vi "test tool call default arguments.vi"(8 "error in (no error)":errorcluster) -> (0 "error out":errorcluster, 3 "body":string)   [LabVIEW 2020, in "MCP Server tests.lvlib"]
doc: "arguments is optional in tools/call. Without it the tool runs with the default values of its inputs: fake_tool_add answers with the sum 0, and the answer is a result, not an error."
uses:
  MCP Server tests.lvlib
  <vilib>/addons/_JKI Toolkits/Caraya/classes/Test/Test.lvclass
  <vilib>/JDP Science/JSONtext/JSONtext.lvlib
  a69b8a6d-5d8a-435b-aaad-afb045a32dc0.vi
  <vilib>/addons/_JKI Toolkits/Caraya/classes/Assert/Assert.lvclass
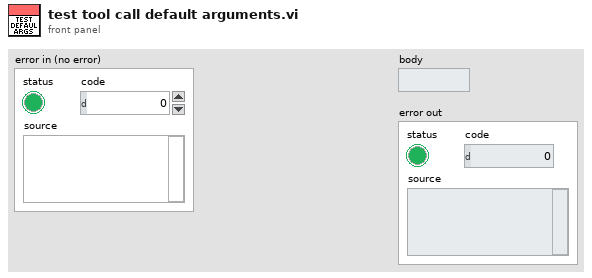
[diagram p1: front panel]
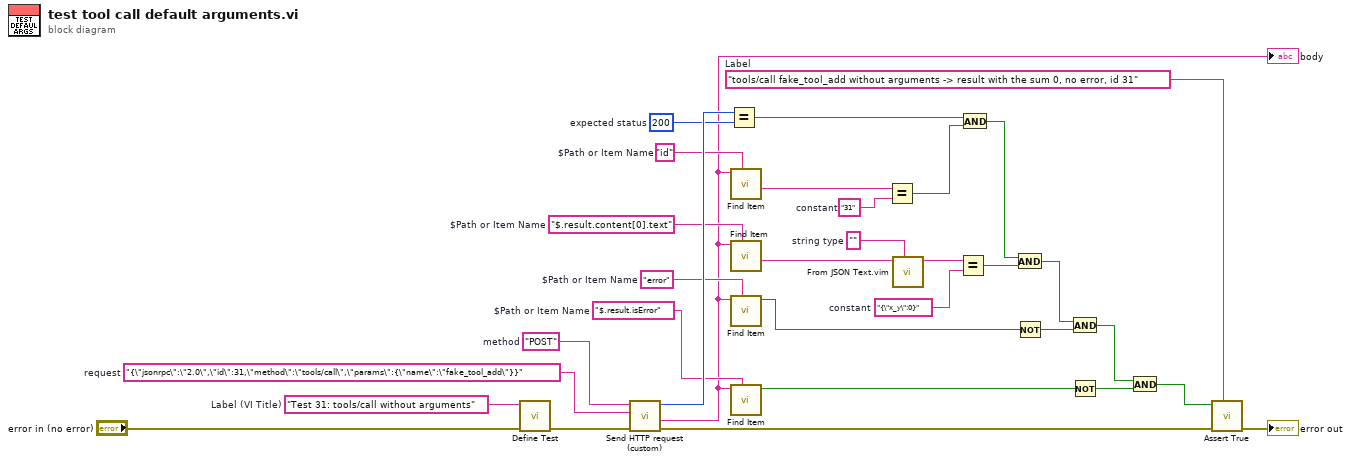
[diagram p0: block diagram]
diagram:
  w3 = "tools/call fake_tool_add without arguments -> result with the sum 0, no error, id 31"  # Label
  w16 = "{\"x_y\":0}"  # constant
  w18 = ""  # string type
  w20 = "31"  # constant
  w22 = "$.result.isError"  # $Path or Item Name
  w23 = "error"  # $Path or Item Name
  w24 = "$.result.content[0].text"  # $Path or Item Name
  w25 = "id"  # $Path or Item Name
  w26 = 200  # expected status
  w29 = "{\"jsonrpc\":\"2.0\",\"id\":31,\"method\":\"tools/call\",\"params\":{\"name\":\"fake_tool_add\"}}"  # request
  w30 = "POST"  # method
  w32 = "Test 31: tools/call without arguments"  # Label (VI Title)
  n1 = call <vilib>:"Define Test.vi"("error in (no error)"="error in (no error)", "Label (VI Title)"=w32) -> ("error out"=w28:errorcluster)  [unwired: 8 in, 1 out]
  n2 = call "Send HTTP request (custom).vi"("error in (no error)"=w28, "request"=w29, "method"=w30) -> ("error out"=w4:errorcluster, "response"=w2:string, "status code"=w27:i32)  [unwired: 5 in, 1 out]
  "body" <- w2
  n3 = Equal?(x=w27, y=w26) -> (x = y?=w13:bool)
  n4 = call <vilib>:"Find Item.vi"("$Path or Item Name"=w25, "JSON"=w2) -> ("<JSON>"=w21:string)  [unwired: 6 in, 3 out]
  n5 = call <vilib>:"Find Item.vi"("$Path or Item Name"=w24, "JSON"=w2) -> ("<JSON>"=w19:string)  [unwired: 6 in, 3 out]
  n6 = call <vilib>:"Find Item.vi"("$Path or Item Name"=w23, "JSON"=w2) -> ("Found"=w15:bool)  [unwired: 6 in, 3 out]
  n7 = call <vilib>:"Find Item.vi"("$Path or Item Name"=w22, "JSON"=w2) -> ("Found"=w14:bool)  [unwired: 6 in, 3 out]
  n8 = Equal?(x=w21, y=w20) -> (x = y?=w12:bool)
  n9 = call "From JSON Text.vim"("Data Type and Default Value"=w18, "JSON"=w19) -> ("Data out"=w17:string)  [unwired: 8 in, 1 out]
  n10 = Equal?(x=w17, y=w16) -> (x = y?=w10:bool)
  n11 = And(x=w13, y=w12) -> (x .and. y?=w11:bool)
  n12 = And(x=w11, y=w10) -> (x .and. y?=w9:bool)
  n13 = Not(x=w15) -> (.not. x?=w8:bool)
  n14 = And(x=w9, y=w8) -> (x .and. y?=w7:bool)
  n15 = Not(x=w14) -> (.not. x?=w6:bool)
  n16 = And(x=w7, y=w6) -> (x .and. y?=w5:bool)
  n17 = call <vilib>:"Assert True.vi"("Label"=w3, "error in (no error)"=w4, "True?"=w5) -> ("error out"=→"error out":errorcluster)  [unwired: 7 in, 1 out]
